vi "rename channel test.vi"() -> (0 "no err":errorcluster, 3 "rename success":bool)   [LabVIEW 2014, in "TEC tests.lvlib"]
uses:
  TEC tests.lvlib
  configuration/TEC configuration.lvclass/TEC configuration.ctl
  <vilib>/NI/Tag Bus/tag/tag descriptor.lvclass/tag descriptor.ctl
  configuration/Write channels.vi
  configuration/TEC configuration.lvclass
  <vilib>/NI/Tag Bus/tag/tag descriptor.lvclass
  <vilib>/NI/Configuration Framework/serializable configuration/NISE_CEF_serializable configuration.lvclass
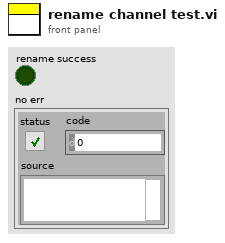
[diagram p1: front panel]
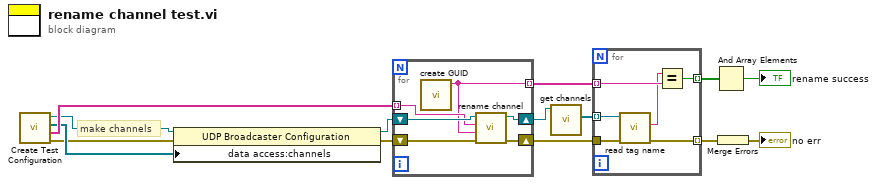
[diagram p0: block diagram]
diagram:
  # "make channels"
  n1 = call "Create Test Configuration.vi"() -> ("error out"=w4:errorcluster, "Channel Names"=w7:string[], "Array"=w6:refnum<class "TBM channel.lvclass">[], "TEC configuration out"=w5:refnum<class "TEC configuration.lvclass">)  [unwired: 8 in]
  n2 = property class="UDP Broadcaster Configuration"(reference=w5, error in=w4, "data access:channels"=w6) -> (reference out=w8:refnum<class "TEC configuration.lvclass">, error out=w9:errorcluster)
  n3 = for {
    tunnel: w7 -> [w16] mode=indexing
    shift-right: [w17] -> w14
    shift-left: w8 -> [w20]
    shift-right: [w18] -> w3
    shift-left: w9 -> [w19]
    tunnel: [w15] -> w13 mode=indexing
    n4 = call <vilib>:"create GUID.vi"() -> ("uuid"=w15:string)  [unwired: 10 in, 1 out]
    n5 = call "rename channel.vi"("error in"=w19, "new name"=w15, "old name"=w16, "TEC configuration in"=w20) -> ("error out"=w18:errorcluster, "TEC configuration out"=w17:refnum<class "TEC configuration.lvclass">)  [unwired: 6 in]
  }
  n6 = call-dynamic "get channels.vi"("TEC configuration in"=w14) -> ("channels"=w12:refnum<class "TBM channel.lvclass">[])  [unwired: 9 in, 1 out]
  n7 = for {
    tunnel: w13 -> [w25] mode=indexing
    tunnel: w12 -> [w26] mode=indexing
    tunnel: [w23] -> w11 mode=indexing
    tunnel: w3 -> [w22]
    tunnel: [w21] -> w2 mode=indexing
    n8 = call <vilib>:"read tag name.vi"("error in"=w22, "system tag in"=w26) -> ("error out"=w21:errorcluster, "name"=w24:string)  [unwired: 7 in, 1 out]
    n9 = Equal?(x=w24, y=w25) -> (x = y?=w23:bool)
  }
  n10 = And Array Elements(Boolean array=w11) -> (logical AND=→"rename success":bool)
  n11 = Merge Errors(w2) -> (→"no err":errorcluster)
